vi "_ConvertTextSettingsToLvText.vi"(11 "TextSettings":T1={"Desired Font"="Application Font", "Strikeout?"=FALSE, "Italic?"=FALSE, "Underline?"=FALSE, "Outline?"=FALSE, "Shadow?"=FALSE, "Bold?"=FALSE, "Size"=12}) -> (1 "alignment":T2, 2 "desired font":T4(ring)=enum."Application Font", 3 "[user-specified font]":T3)   [LabVIEW 2020, in "OpenLvVision_Overlays.lvlib"]
uses:
  OpenLvVision_Overlays.lvlib
  TypeDefs/TextSettings.ctl
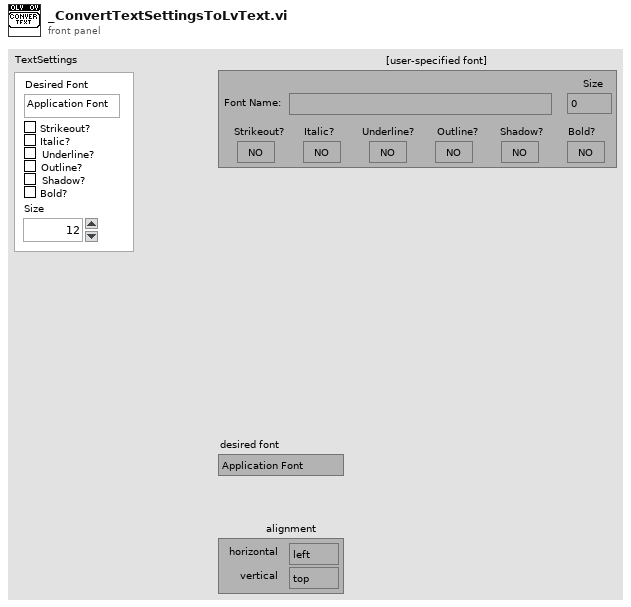
[diagram p1: front panel]
types:
  T1 = typedef "OpenLvVision_Overlays.lvlib/TextSettings.ctl" = cluster{"Desired Font":string, "Strikeout?":bool, "Italic?":bool, "Underline?":bool, "Outline?":bool, "Shadow?":bool, "Bold?":bool, "Size":i32}
  T2 = cluster{"horizontal":enum16{"left", "center", "right"}, "vertical":enum16{"top", "center", "bottom"}}
  T3 = cluster{"Font Name:":string, "Size":i16, "Strikeout?":bool, "Italic?":bool, "Underline?":bool, "Outline?":bool, "Shadow?":bool, "Bold?":bool}
  T4 = enum16{"User-specified Font", "Application Font", "System Font", "Dialog Font"}
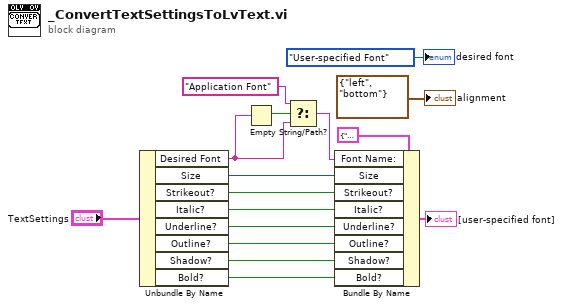
[diagram p0: block diagram]
diagram:
  n1 = Unbundle By Name("TextSettings") -> ("Desired Font"=w1:string, "Size"=w14:i32, "Strikeout?"=w13:bool, "Italic?"=w12:bool, "Underline?"=w11:bool, "Outline?"=w10:bool, "Shadow?"=w9:bool, "Bold?"=w8:bool)
  n2 = Empty String/Path?(string/path=w1) -> (empty?=w4:bool)
  n3 = Select(t="Application Font", s=w4, f=w1) -> (s? t:f=w3:string)
  n4 = Bundle By Name(cluster=T3 {"Font Name:"="", "Size"=0, "Strikeout?"=FALSE, "Italic?"=FALSE, "Underline?"=FALSE, "Outline?"=FALSE, "Shadow?"=FALSE, "Bold?"=FALSE} ("[user-specified font]"), "Font Name:"=w3, "Size"=w14, "Strikeout?"=w13, "Italic?"=w12, "Underline?"=w11, "Outline?"=w10, "Shadow?"=w9, "Bold?"=w8) -> (→"[user-specified font]":T3)
  "desired font" <- T4."User-specified Font" ("desired font")
  "alignment" <- T2 {"horizontal"=enum."left", "vertical"=enum."bottom"} ("alignment(left, top)")
